vi "LatchBooleanKeyboardSimulation_Tests.vi"(11 "error in":errorcluster) -> (15 "error out":errorcluster)   [LabVIEW 2016, in "DronaTest.lvlib"]
uses:
  DronaTest.lvlib
  APIs/Stimulus/ControlValue/ValueSignalLatchBooleanString.vi
  APIs/Assert/AssertControlValue/Equal.vi
  <vilib>/addons/_JKI Toolkits/Caraya/classes/Test/Test.lvclass
  Drona.lvlib
  APIs/Assert/AssertControlValue/AssertControlValue.lvlib
  APIs/Stimulus/ControlValue/ControlValue.lvlib
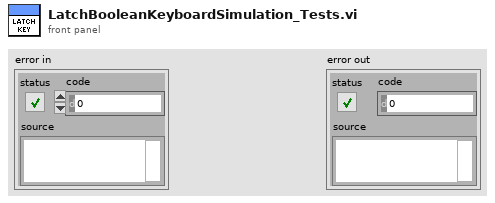
[diagram p1: front panel]
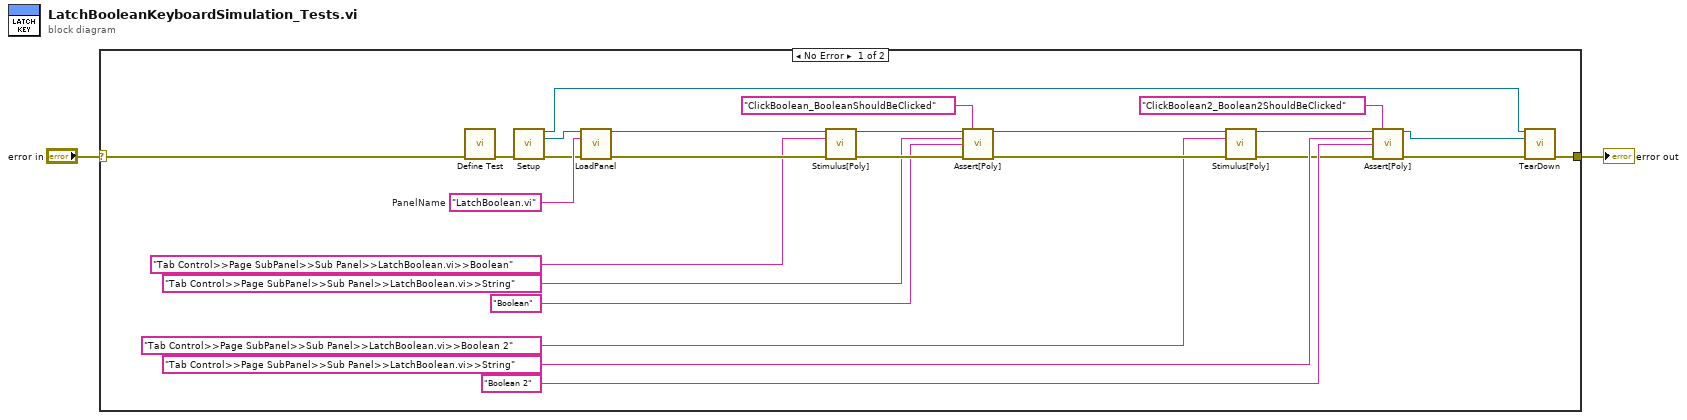
[diagram p0: block diagram]
diagram:
  n1 = case shown="No Error" "error in" {
    selector: "error in" -> [w27 w28]
    tunnel: [w7 w28] -> w1
    frame No Error {
      w26 = "LatchBoolean.vi"  # PanelName
      n2 = call <vilib>:"Define Test.vi"("error in (no error)"=w27) -> ("error out"=w8:errorcluster)  [unwired: 9 in, 1 out]
      n3 = call "Setup.vi"("error in (no error)"=w8) -> ("Application Ref"=w6:refnum<vi>, "VI out"=w4:refnum<vi>, "error out"=w5:errorcluster)  [unwired: 12 in]
      n4 = call "LoadPanel.vi"("VI in"=w4, "Item Name"=w26, "error in (no error)"=w5) -> ("VI out"=w24:refnum<vi>, "error out"=w11:errorcluster)  [unwired: 11 in]
      n5 = call-poly "Stimulus[Poly].vi"("VI Reference In"=w24, "Control Path"="Tab Control>>Page SubPanel>>Sub Panel>>LatchBoolean.vi>>Boolean", "error in"=w11) -> ("VI Reference Out"=w23:refnum<vi>, "error out"=w25:errorcluster)  [unwired: 11 in]
      n6 = call-poly "Assert[Poly].vi"("VI Reference In"=w23, "Test Label"="ClickBoolean_BooleanShouldBeClicked" ("string"), "Control Path"="Tab Control>>Page SubPanel>>Sub Panel>>LatchBoolean.vi>>String", "Control Value"="Boolean" ("Control Path"), "Error In"=w25) -> ("VI Reference Out"=w13:refnum<vi>, "Error Out"=w14:errorcluster)  [unwired: 8 in, 1 out]
      n7 = call-poly "Stimulus[Poly].vi"("VI Reference In"=w13, "Control Path"="Tab Control>>Page SubPanel>>Sub Panel>>LatchBoolean.vi>>Boolean 2", "error in"=w14) -> ("VI Reference Out"=w16:refnum<vi>, "error out"=w15:errorcluster)  [unwired: 11 in]
      n8 = call-poly "Assert[Poly].vi"("VI Reference In"=w16, "Test Label"="ClickBoolean2_Boolean2ShouldBeClicked" ("string"), "Control Path"="Tab Control>>Page SubPanel>>Sub Panel>>LatchBoolean.vi>>String", "Control Value"="Boolean 2" ("Control Path"), "Error In"=w15) -> ("VI Reference Out"=w3:refnum<vi>, "Error Out"=w12:errorcluster)  [unwired: 8 in, 1 out]
      n9 = call "TearDown.vi"("Application Ref"=w6, "VI in"=w3, "error in (no error)"=w12) -> ("error out"=w7:errorcluster)  [unwired: 12 in]
    }
    frame Error {
    }
  }
  "error out" <- w1
